vi "Load_Icons.vi"(11 "Error In":errorcluster) -> (15 "Error Out":errorcluster)   [LabVIEW 2026, in "Core.lvlib"]
doc: "This VI loads icons from a folder to to the specified controls. The images must be the same name as the control, and in png format."
uses:
  Core.lvlib
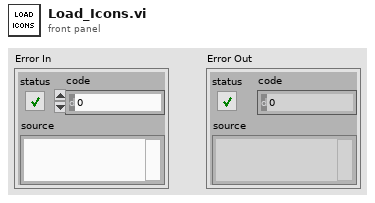
[diagram p1: front panel]
types:
  T1 = typedef "imagedata.ctl" = cluster{"image type":i32, "image depth":i32, "image":u8[], "mask":u8[], "colors":u32[], "Rectangle":cluster{"left":i16, "top":i16, "right":i16, "bottom":i16}}
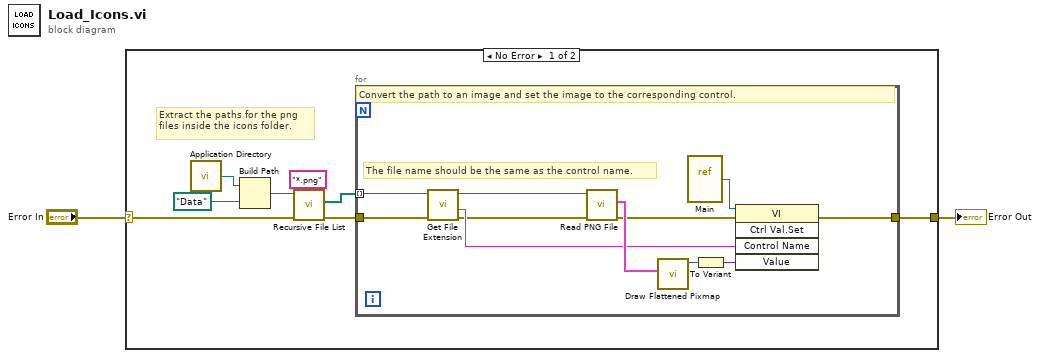
[diagram p0: block diagram]
diagram:
  n1 = case shown="No Error" "Error In" {
    selector: "Error In" -> [w4 w22]
    tunnel: [w10 w22] -> w2
    frame No Error {
      # "Extract the paths for the png files inside the icons folder."
      n2 = call <vilib>:"Application Directory.vi"() -> ("Application Directory"=w7:path)
      n3 = Build Path(base path=w7, name or relative path=path "Data") -> (appended path=w9:path)
      n4 = call <vilib>:"Recursive File List.vi"("pattern"="*.png", "error in (no error)"=w4, "Folder Path"=w9) -> ("error out"=w3:errorcluster, "All Files in Dir"=w6:path[])  [unwired: 4 in, 3 out]
      n5 = for {
        tunnel: w6 -> [w20] mode=indexing
        tunnel: w3 -> [w16]
        tunnel: [w12] -> w10
        # "The file name should be the same as the control name."
        # "Convert the path to an image and set the image to the corresponding control."
        n6 = call <vilib>:"Get File Extension.vi"("error in (no error)"=w16, "file"=w20) -> ("error out"=w14:errorcluster, "filename without extension"=w19:string, "dup file"=w15:path)  [unwired: 5 in, 2 out]
        n7 = call <vilib>:"Read PNG File.vi"("error in (no error)"=w14, "path to PNG file"=w15) -> ("error out"=w13:errorcluster, "image data"=w21:T1)  [unwired: 7 in, 1 out]
        n8 = call <vilib>:"Draw Flattened Pixmap.vi"("image data"=w21) -> ("new picture"=w18:picture)  [unwired: 8 in]
        n9 = vi-ref "Main.vi"() -> (w11:refnum<vi>)
        n10 = To Variant(anything=w18) -> (Variant=w17:variant)
        n11 = invoke class="VI" method="Ctrl Val.Set"(reference=w11, error in=w13, "Control Name"=w19, "Value"=w17) -> (error out=w12:errorcluster)  [unwired: 1 in, 4 out]
      }
    }
    frame Error {
    }
  }
  "Error Out" <- w2
